vi "Create New Handler.vi"(7 "Handler type":refnum<class "Handler.lvclass">, 8 "error in (no error)":errorcluster, 10 "Name":string, 11 "Level":T1(ring)) -> (0 "error out":errorcluster, 3 "Handler":refnum<class "Handler.lvclass">)   [LabVIEW 2017, in "Error Log.lvlib" / "Handler.lvclass"]
doc: "Creates a new <b>Handler</b> nammed <b>Name</b> to log message with severity equal or higher than <b>Level</b>."
uses:
  Handler.lvclass
  Handler.lvclass/Handler.ctl
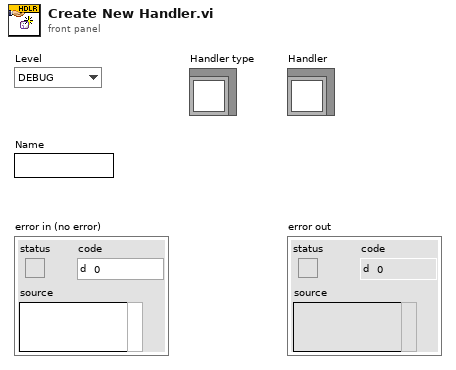
[diagram p1: front panel]
types:
  T1 = enum16{"DEBUG", "INFO", "WARNING", "ERROR", "CRITICAL"}
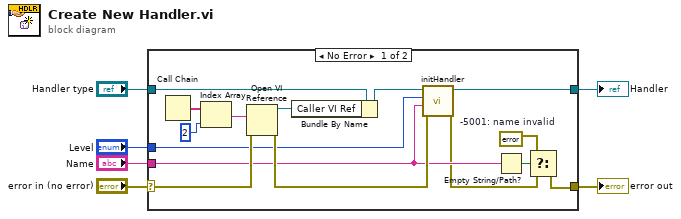
[diagram p0: block diagram]
diagram:
  n1 = case shown="No Error" "error in (no error)" {
    selector: "error in (no error)" -> [w14 w23]
    tunnel: [w7 w23] -> w5
    tunnel: [w15 w22] -> w3
    tunnel: "Handler type" -> [w17 w22]
    tunnel: "Level" -> [w12 _]
    tunnel: "Name" -> [w11 _]
    frame No Error {
      w9 = errorcluster {"status"=TRUE, "code"=5001, "source"="Handler Name is invalid"}  # -5001: name invalid
      n2 = Call Chain() -> (call chain=w20:string[])
      n3 = Index Array(array=w20, index=2 ("Index")) -> (element=w21:string)
      n4 = Open VI Reference(vi path=w21, error in (no error)=w14) -> (vi reference=w18:refnum<vi>, error out=w13:errorcluster)  [unwired: 4 in]
      n5 = Bundle By Name(cluster=w17, "Caller VI Ref"=w18) -> (w16:refnum<class "Handler.lvclass">)
      n6 = call-dynamic "initHandler.vi"("error in (no error)"=w13, "Name"=w11, "Level"=w12, "Handler in"=w16) -> ("error out"=w8:errorcluster, "Handler out"=w15:refnum<class "Handler.lvclass">)  [unwired: 6 in]
      n7 = Empty String/Path?(string/path=w11) -> (empty?=w10:bool)
      n8 = Select(t=w9, s=w10, f=w8) -> (s? t:f=w7:errorcluster)
    }
    frame Error {
    }
  }
  "error out" <- w5
  "Handler" <- w3
